vi "calculate Possible Search Line Frequency.vi"(10 "Marker Search Freq (Hz)":T1 {"Right Limit" format="%#_6p"; "Left Limit" format="%#_6p"}, 11 "Start/Stop Frequency(Hz)":T2 {"Stop" format="%#_6p"; "Start" format="%#_6p"}) -> (3 "Calculated Marker Search Freq (Hz)":T1 {"Right Limit" format="%#_6p"; "Left Limit" format="%#_6p"})   [LabVIEW 2023, in "Spectrum Analyzer.lvlib"]
uses:
  Spectrum Analyzer.lvlib
  TYPE DEFINITION/TYPE Start and Stop Frequency.ctl
  TYPE DEFINITION/TYPE Marker Search Limit Set.ctl
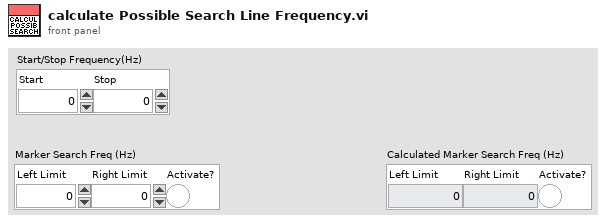
[diagram p1: front panel]
types:
  T1 = typedef "Spectrum Analyzer.lvlib/TYPE Marker Search Limit Set.ctl" = cluster{"Left Limit":dbl, "Right Limit":dbl, "Activate?":bool}
  T2 = typedef "Spectrum Analyzer.lvlib/TYPE Start and Stop Frequency.ctl" = cluster{"Start":dbl, "Stop":dbl}
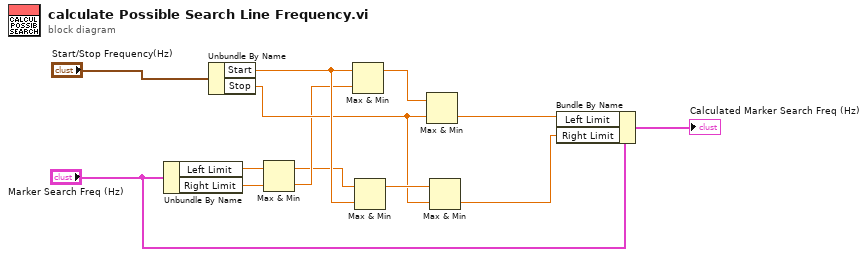
[diagram p0: block diagram]
diagram:
  n1 = Unbundle By Name("Marker Search Freq (Hz)") -> ("Left Limit"=w4:dbl, "Right Limit"=w3:dbl)
  n2 = Unbundle By Name("Start/Stop Frequency(Hz)") -> ("Start"=w11:dbl, "Stop"=w9:dbl)
  n3 = Max & Min(x=w4, y=w3) -> (max(x,y)=w1:dbl, min(x,y)=w2:dbl)
  n4 = Max & Min(x=w11, y=w2) -> (max(x,y)=w12:dbl)  [unwired: 1 out]
  n5 = Max & Min(x=w1, y=w11) -> (max(x,y)=w10:dbl)  [unwired: 1 out]
  n6 = Max & Min(x=w12, y=w9) -> (min(x,y)=w7:dbl)  [unwired: 1 out]
  n7 = Max & Min(x=w10, y=w9) -> (min(x,y)=w6:dbl)  [unwired: 1 out]
  n8 = Bundle By Name(cluster="Marker Search Freq (Hz)", "Left Limit"=w7, "Right Limit"=w6) -> (→"Calculated Marker Search Freq (Hz)":T1)
